vi "Func - Load Functions.vi"(6 "error in":errorcluster, 7 "test arg num (F)":bool, 8 "Array of func names":string[](array[string]), 9 "List of func names":string) -> (0 "error out":errorcluster, 1 "error message":string, 2 "loaded functions":string[](array[string]))   [LabVIEW 2021]
doc: "This VI explicitly loads FuncVIs into memory. Loading a FuncVI before its corresponding function is called during script execution reduces the execution time of the first call. Refer to the VI help for more details.\n\nPass function names to either the <b>Array of func names</b> control or the <b>List of func names</b> control. Note that this VI recognizes function names, not FuncVI names. Therefore, to load a FuncVI, you must specify the name of the corresponding function.\n\n::: CalcExpress Toolkit :::\nCopyright (c) 2000-2026 Konstantin Shifershteyn. All rights reserved."
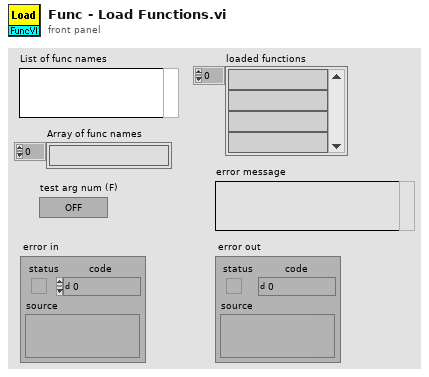
[diagram p1: front panel]
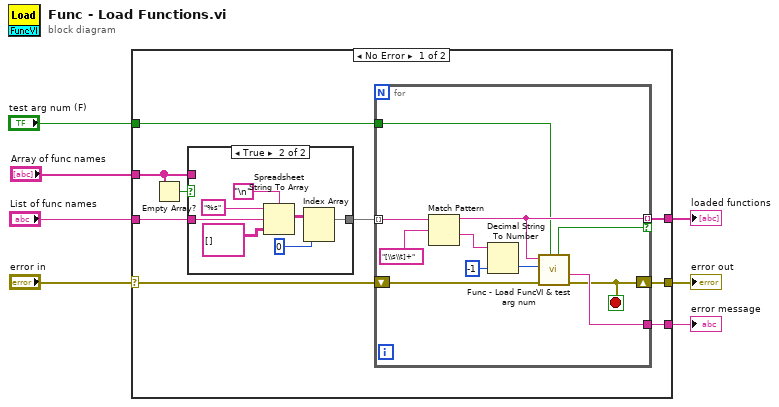
[diagram p0: block diagram]
diagram:
  n1 = case shown="No Error" "error in" {
    selector: "error in" -> [w16 w36]
    tunnel: [w15 w36] -> w4
    tunnel: "test arg num (F)" -> [w14 _]
    tunnel: [w13 _] -> w5
    tunnel: [w12 _] -> w3
    tunnel: "Array of func names" -> [w8 _]
    tunnel: "List of func names" -> [w11 _]
    frame No Error {
      n2 = Empty Array?(array=w8) -> (empty?=w9:bool)
      n3 = case shown="True" w9 {
        tunnel: [w17 w20] -> w10
        tunnel: w8 -> [w17 _]
        tunnel: w11 -> [_ w22]
        frame False {
        }
        frame True {
          n4 = Spreadsheet String To Array(delimiter (Tab)="\n", format string="%s", spreadsheet string=w22, array type (2D Dbl)=string[][] []) -> (array=w21:string[][])
          n5 = Index Array(array=w21, index (col)=0) -> (element=w20:string[])  [unwired: 1 in]
        }
      }
      n6 = for {
        tunnel: [w31] -> w13 mode=indexing if=w29
        tunnel: w10 -> [w32] mode=indexing
        tunnel: [w28] -> w12
        shift-right: [w26] -> w15
        shift-left: w16 -> [w27]
        tunnel: w14 -> [w25]
        stop <- w26 stop-if-true
        n7 = Match Pattern(string=w32, regular expression="[\\s\\t]+") -> (before substring=w31:string, after substring=w33:string)  [unwired: 1 in, 2 out]
        n8 = Decimal String To Number(string=w33, default (0L)=-1) -> (number=w30:i32)  [unwired: 1 in, 1 out]
        n9 = call "Func - Load FuncVI & test arg num.vi"("test arg num"=w25, "error in"=w27, "arg num"=w30, "func name"=w31) -> ("error out"=w26:errorcluster, "error message"=w28:string, "loaded"=w29:bool)  [unwired: 2 in, 1 out]
      }
    }
    frame Error {
    }
  }
  "error out" <- w4
  "loaded functions" <- w5
  "error message" <- w3
